vi "Send Message.vi"(8 "error in (no error)":errorcluster, 10 "Message":T1={"Command"="", "Data"=variant(string ""), "ID"="", "error"={"status"=FALSE, "code"=0, "source"=""}}, 11 "RemoteControl.ZMQ in":refnum<class "RemoteControl.ZMQ.lvclass">) -> (0 "error out":errorcluster, 3 "RemoteControl.ZMQ out":refnum<class "RemoteControl.ZMQ.lvclass">)   [LabVIEW 2019, in "RemoteControl.ZMQ.lvlib" / "RemoteControl.ZMQ.lvclass"]
uses:
  RemoteControl.ZMQ.lvclass
  C:/Program Files/National Instruments/LabVIEW 2019/user.lib/LevyLab/RemoteControl/RemoteControl/RemoteControl.lvclass
  <userlib>/LevyLab/RemoteControl/RemoteControl/Typedefs/Message--Cluster.ctl
  RemoteControl.ZMQ.lvclass/RemoteControl.ZMQ.ctl
  <userlib>/LevyLab/RemoteControl/RemoteControl/RemoteControl.lvclass/RemoteControl.ctl
  <vilib>/PRIrvin/JSON-RPC/JSON-RPC.lvlib
  <vilib>/addons/zeromq/zmq_socket.lvclass
  <userlib>/LevyLab/RemoteControl/RemoteControl/RemoteControl.lvclass
  C:/Program Files/National Instruments/LabVIEW 2019/vi.lib/JKI/JKI SMO/SMO/SMO.lvclass
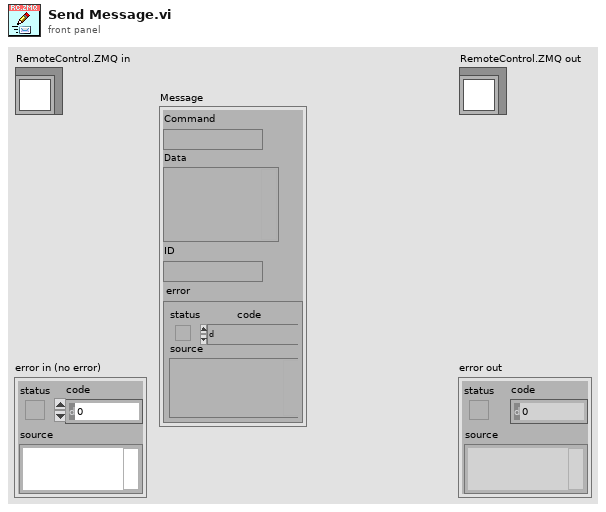
[diagram p1: front panel]
types:
  T1 = typedef "RemoteControl.lvlib/RemoteControl.lvclass/Message--Cluster.ctl" = cluster{"Command":string, "Data":variant, "ID":string, "error":errorcluster}
  T2 = typedef "zeromq.lvlib/socket_type.ctl" = enum8{"ZMQ_PAIR", "ZMQ_PUB", "ZMQ_SUB", "ZMQ_REQ", "ZMQ_REP", "ZMQ_DEALER", "ZMQ_ROUTER", "ZMQ_PULL", "ZMQ_PUSH", "ZMQ_XPUB", "ZMQ_XSUB", "ZMQ_STREAM", "ZMQ_SERVER", "ZMQ_CLIENT", "ZMQ_RADIO", "ZMQ_DISH", "ZMQ_GATHER", "ZMQ_SCATTER", "ZMQ_DGRAM"}
  T3 = cluster{"Command":string, "Data":variant, "ID":string}
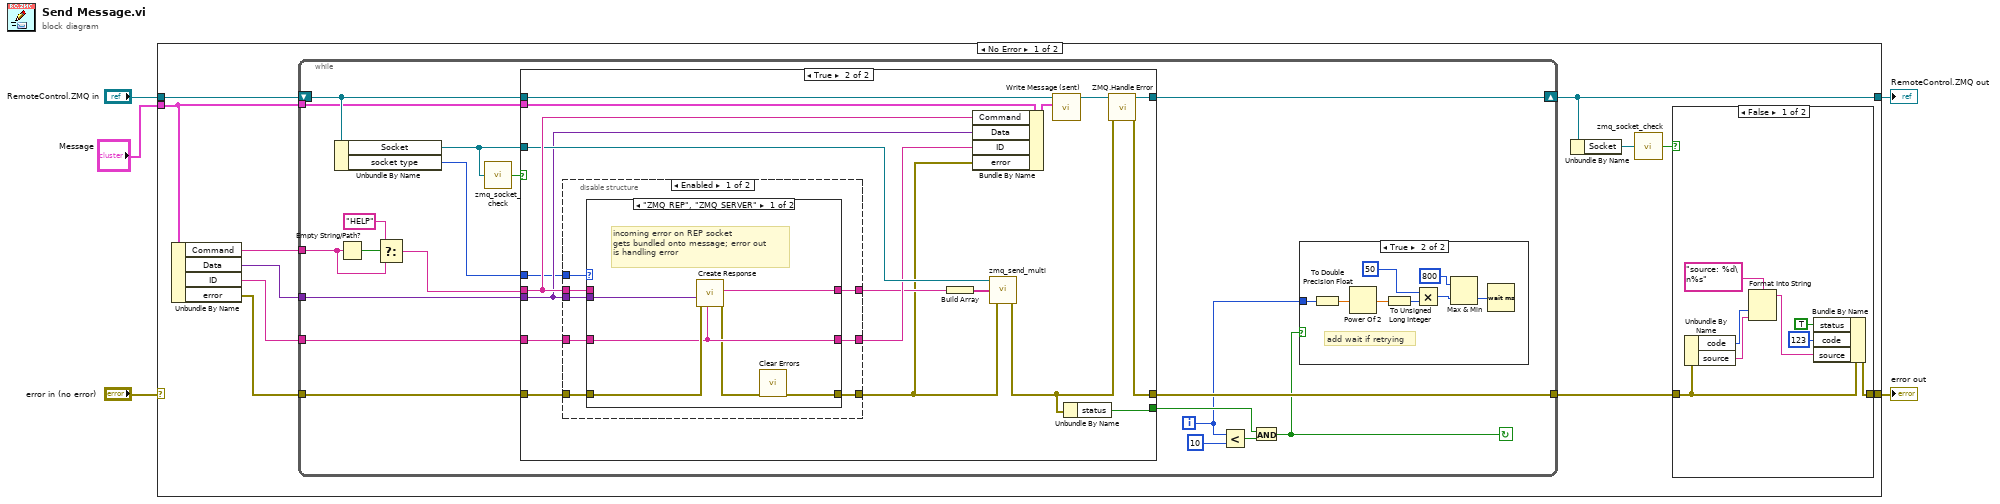
[diagram p0: block diagram]
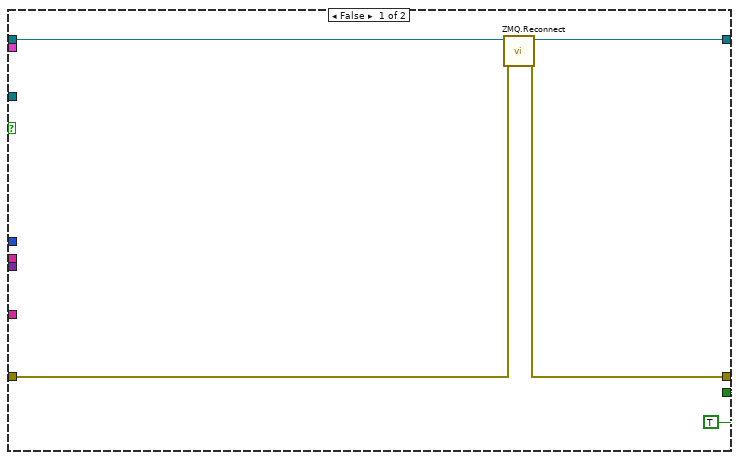
[diagram p2: hidden frame]
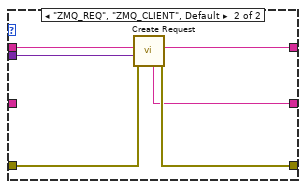
[diagram p3: hidden frame]
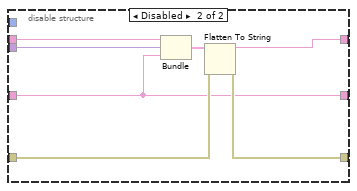
[diagram p4: hidden frame]
diagram:
  n1 = case shown="No Error" "error in (no error)" {
    selector: "error in (no error)" -> [_ w104]
    tunnel: [w10 w103] -> w5
    tunnel: [w7 w104] -> w4
    tunnel: "RemoteControl.ZMQ in" -> [w16 w103]
    tunnel: "Message" -> [w12 _]
    frame No Error {
      n2 = Unbundle By Name(w12) -> ("Command"=w15:string, "Data"=w14:variant, "ID"=w13:string, "error"=w11:errorcluster)
      n3 = while {
        tunnel: w15 -> [w30]
        tunnel: w13 -> [w33]
        tunnel: w14 -> [w26]
        shift-right: [w31] -> w10
        shift-left: w16 -> [w32]
        tunnel: w11 -> [w29]
        tunnel: [w24] -> w6
        tunnel: w12 -> [w27]
        i -> [w17]
        stop <- w19 continue-if-true
        n4 = Unbundle By Name(w32) -> ("Socket"=w23:refnum<class "zmq_socket.lvclass">, "socket type"=w25:T2)
        n5 = Empty String/Path?(string/path=w30) -> (empty?=w34:bool)
        n6 = Select(t="HELP", s=w34, f=w30) -> (s? t:f=w28:string)
        n7 = call <vilib>:"zmq_socket_check.vi"("socket in"=w23) -> ("valid?"=w22:bool)
        n8 = case shown="True" w22 {
          tunnel: w33 -> [_ w58]
          tunnel: w32 -> [w39 w56]
          tunnel: [w38 w54] -> w31
          tunnel: w29 -> [w36 w53]
          tunnel: w28 -> [_ w52]
          tunnel: w27 -> [_ w51]
          tunnel: w23 -> [_ w48]
          tunnel: w26 -> [_ w44]
          tunnel: w25 -> [_ w43]
          tunnel: [TRUE w41] -> w18
          tunnel: [w37 w42] -> w24
          frame False {
            n9 = call "ZMQ.Reconnect.vi"("error in (no error)"=w36, "RemoteControl.ZMQ in"=w39) -> ("error out"=w37:errorcluster, "RemoteControl.ZMQ out"=w38:refnum<class "RemoteControl.ZMQ.lvclass">)  [unwired: 8 in]
          }
          frame True {
            n10 = disable-structure shown="Enabled" {
              disable-tunnel: w44 -> [w66 w81]
              disable-tunnel: w52 -> [w65 w82]
              disable-tunnel: [w64 w79] -> w46
              disable-tunnel: w53 -> [w63 w84]
              disable-tunnel: [w62 w83] -> w45
              disable-tunnel: w43 -> [w61 _]
              disable-tunnel: w58 -> [w59 w80]
              disable-tunnel: [w60 w80] -> w47
              frame Enabled {
                n11 = case shown="\"ZMQ_REP\", \"ZMQ_SERVER\"" w61 {
                  tunnel: w65 -> [_ w74]
                  tunnel: w66 -> [w69 w75]
                  tunnel: [w70 w76] -> w64
                  tunnel: w63 -> [w72 w78]
                  tunnel: [w67 w77] -> w62
                  tunnel: w59 -> [w71 _]
                  tunnel: [w71 w73] -> w60
                  frame "ZMQ_REP", "ZMQ_SERVER" {
                    # "incoming error on REP socket\ngets bundled onto message; error out\nis handling error"
                    n12 = call <vilib>:"Create Response.vi"("id"=w71, "error in (no error)"=w72, "result"=w69) -> ("error out"=w68:errorcluster, "<JSON> Response"=w70:string)  [unwired: 7 in]
                    n13 = call <vilib>:"Clear Errors.vi"("error in (no error)"=w68) -> ("error out"=w67:errorcluster)  [unwired: 5 in, 1 out]
                  }
                  frame "ZMQ_REQ", "ZMQ_CLIENT", Default {
                    n14 = call <vilib>:"Create Request.vi"("error in (no error)"=w78, "params"=w75, "method"=w74) -> ("error out"=w77:errorcluster, "<JSON> Requests"=w76:string, "IDs"=w73:string)  [unwired: 6 in]
                  }
                }
              }
              frame Disabled {
                n15 = Bundle("Command"=w82, "Data"=w81, "ID"=w80) -> (w85:T3)  [unwired: 1 in]
                n16 = Flatten To String(anything=w85, error in (no error)=w84) -> (data string=w79:string, error out=w83:errorcluster)  [unwired: 2 in, 1 out]
              }
            }
            n17 = Build Array(w46) -> (w57:string[])
            n18 = Bundle By Name(cluster=w51, "Command"=w52, "Data"=w44, "ID"=w47, "error"=w45) -> (w50:T1)
            n19 = call <vilib>:"zmq_send_multi.vi"("error in"=w45, "parts"=w57, "socket in"=w48) -> ("error out"=w49:errorcluster)  [unwired: 1 in, 1 out]
            n20 = call <userlib>:"Write Message (sent).vi"("Message"=w50, "RemoteControl in"=w56) -> ("RemoteControl out"=w55:refnum<class "RemoteControl.ZMQ.lvclass">)  [unwired: 9 in]
            n21 = Unbundle By Name(w49) -> ("status"=w41:bool)
            n22 = call "ZMQ.Handle Error.vi"("error in (no error)"=w49, "RemoteControl.ZMQ in"=w55) -> ("error out"=w42:errorcluster, "RemoteControl.ZMQ out"=w54:refnum<class "RemoteControl.ZMQ.lvclass">)  [unwired: 8 in]
          }
        }
        n23 = Less?(x=w17, y=10) -> (x < y?=w21:bool)
        n24 = And(x=w18, y=w21) -> (x .and. y?=w19:bool)
        n25 = case shown="True" w19 {
          tunnel: w17 -> [_ w89]
          frame False {
          }
          frame True {
            # "add wait if retrying"
            n26 = To Double Precision Float(number=w89) -> (double precision float=w90:dbl)
            n27 = Power Of 2(x=w90) -> (2^x=w93:dbl)
            n28 = To Unsigned Long Integer(number=w93) -> (unsigned 32bit integer=w91:u32)
            n29 = Multiply(x=u32 50 ("milliseconds to wait"), y=w91) -> (x*y=w88:u32)
            n30 = Max & Min(x=u32 800 ("upper limit"), y=w88) -> (min(x,y)=w86:u32)  [unwired: 1 out]
            n31 = Wait (ms)(milliseconds to wait=w86) -> ()  [unwired: 1 out]
          }
        }
      }
      n32 = Unbundle By Name(w10) -> ("Socket"=w9:refnum<class "zmq_socket.lvclass">)
      n33 = call <vilib>:"zmq_socket_check.vi"("socket in"=w9) -> ("valid?"=w8:bool)
      n34 = case shown="False" w8 {
        tunnel: [w97 w102] -> w7
        tunnel: w6 -> [w98 w102]
        frame False {
          n35 = Unbundle By Name(w98) -> ("code"=w96:i32, "source"=w95:string)
          n36 = Format Into String(format string="source: %d\n%s", w96, w95) -> (resulting string=w94:string)  [unwired: 2 in, 1 out]
          n37 = Bundle By Name(cluster=w98, "status"=TRUE, "code"=123, "source"=w94) -> (w97:errorcluster)
        }
        frame True {
        }
      }
    }
    frame Error {
    }
  }
  "error out" <- w4
  "RemoteControl.ZMQ out" <- w5
